vi "Get Rx Configuration.vi"(8 "error in":errorcluster, 11 "custom device":T1 format="%.0x") -> (0 "error out":errorcluster, 2 "configuration string out":string, 3 "custom device out":T1 format="%.0x")   [LabVIEW 2020, in "Ballard ARINC 429 Hardware Configuration.lvlib"]
uses:
  Ballard ARINC 429 Hardware Configuration.lvlib
  <vilib>/NI VeriStand/Custom Device API/Custom Device Item Ref.ctl
  Constants.vi
  Scripting/Ballard/Ballard ARINC 429 Scripting.lvlib
  Scripting/ARINC 429/ARINC 429 Scripting.lvlib
  <vilib>/NI VeriStand/Custom Device API/Custom Device API.lvlib
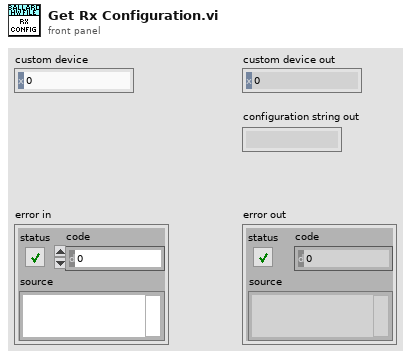
[diagram p1: front panel]
types:
  T1 = typedef "Custom Device API.lvlib/Custom Device Item Ref.ctl" = u64
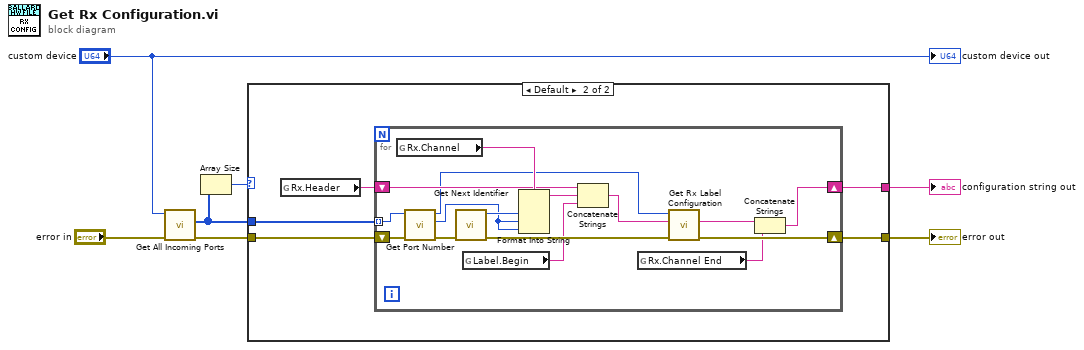
[diagram p0: block diagram]
diagram:
  n1 = call "Get All Incoming Ports.vi"("error in"="error in", "Ballard ARINC 429 custom device in"="custom device") -> ("error out"=w5:errorcluster, "incoming ports"=w2:T1[])  [unwired: 7 in, 1 out]
  n2 = Array Size(array=w2) -> (size(s)=w1:i32)
  n3 = case shown="Default" w1 {
    tunnel: w2 -> [_ w13]
    tunnel: w5 -> [w8 w12]
    tunnel: [_ w11] -> w4
    tunnel: [w8 w10] -> w3
    frame ..0 {
    }
    frame Default {
      n4 = global read "Constants.vi" "Rx.Header"() -> (w9:string)
      n5 = for {
        tunnel: w13 -> [w28] mode=indexing
        shift-right: [w18] -> w10
        shift-left: w12 -> [w29]
        shift-right: [w15] -> w11
        shift-left: w9 -> [w23]
        n6 = global read "Constants.vi" "Rx.Channel"() -> (w26:string)
        n7 = call "Get Port Number.vi"("error in"=w29, "port ref in"=w28) -> ("error out"=w27:errorcluster, "port number"=w24:u16, "port ref out"=w21:T1)  [unwired: 6 in, 1 out]
        n8 = call "Get Next Identifier.vi"("error in"=w27) -> ("error out"=w19:errorcluster, "ID"=w25:u32)  [unwired: 9 in]
        n9 = global read "Constants.vi" "Label.Begin"() -> (w17:string)
        n10 = Format Into String(format string=w26, w25, w24, w24) -> (resulting string=w22:string)  [unwired: 2 in, 1 out]
        n11 = Concatenate Strings(w23, w22, w17) -> (w20:string)
        n12 = global read "Constants.vi" "Rx.Channel End"() -> (w14:string)
        n13 = call "Get Rx Label Configuration.vi"("error in"=w19, "configuration string"=w20, "port ref"=w21) -> ("error out"=w18:errorcluster, "configuration string out"=w16:string)  [unwired: 6 in, 1 out]
        n14 = Concatenate Strings(w16, w14) -> (w15:string)
      }
    }
  }
  "error out" <- w3
  "configuration string out" <- w4
  "custom device out" <- "custom device"
